vi "runDetectionB.vi"(0 "dl in":refnum<class "dl.lvclass">, 1 "batchSIze":i32=1, 2 "convert\nBGR2RGB":enum16{"False", "True"}(ring), 3 "BCHW":u16(ring)=1 items=["False", "True"], 4 "normalizeto255":enum16{"False", "True"}(ring), 5 "error in (no error)":errorcluster) -> (14 "dl out":refnum<class "dl.lvclass">, 15 "runSucc":i32, 16 "bbCounts":i32[](array[numeric]), 17 "maskCounts":i32[](array[numeric]), 19 "error out":errorcluster)   [LabVIEW 2025, in "dl.lvlib" / "dl.lvclass"]
doc: "Run Deep Learning Models – Bounding Box Detection and Segmentation**\n\nInputs:\n- `batchSize`: Number of input images (default: 1).\n- `BGR2RGB`: Convert image color format from BGR to RGB (default: false).\n- `BCHW`: Indicates whether the input is already in BCHW format (default: true).\n- `normalize255`: Normalize pixel values by dividing by 255 (default: false).\n\nOutputs:\n- `runSucc`: Algorithm execution status. `0` indicates success; any other value indicates an error.\n- `bbCounts`: Number of detected bounding boxes per image.\n- `maskCounts`: Number of detected segmentation masks per image."
uses:
  dl.lvclass
  dl.lvclass/dl.ctl
  e74e055a-5232-42f4-a9d8-d9d66c19bc29.vi
  0898d0a7-90d2-4c31-95aa-5e649e2e6c68.vi
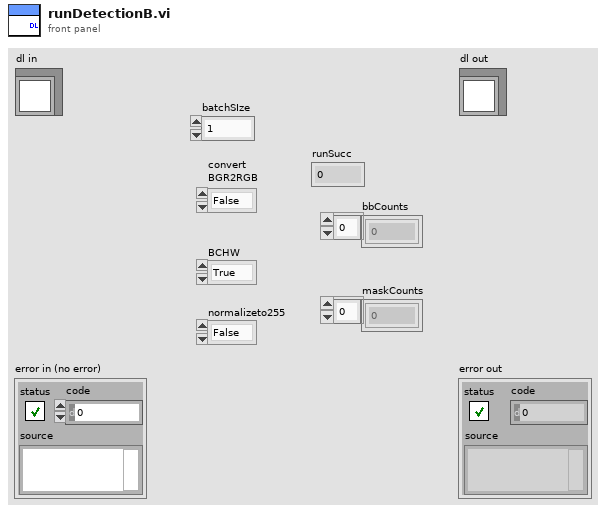
[diagram p1: front panel]
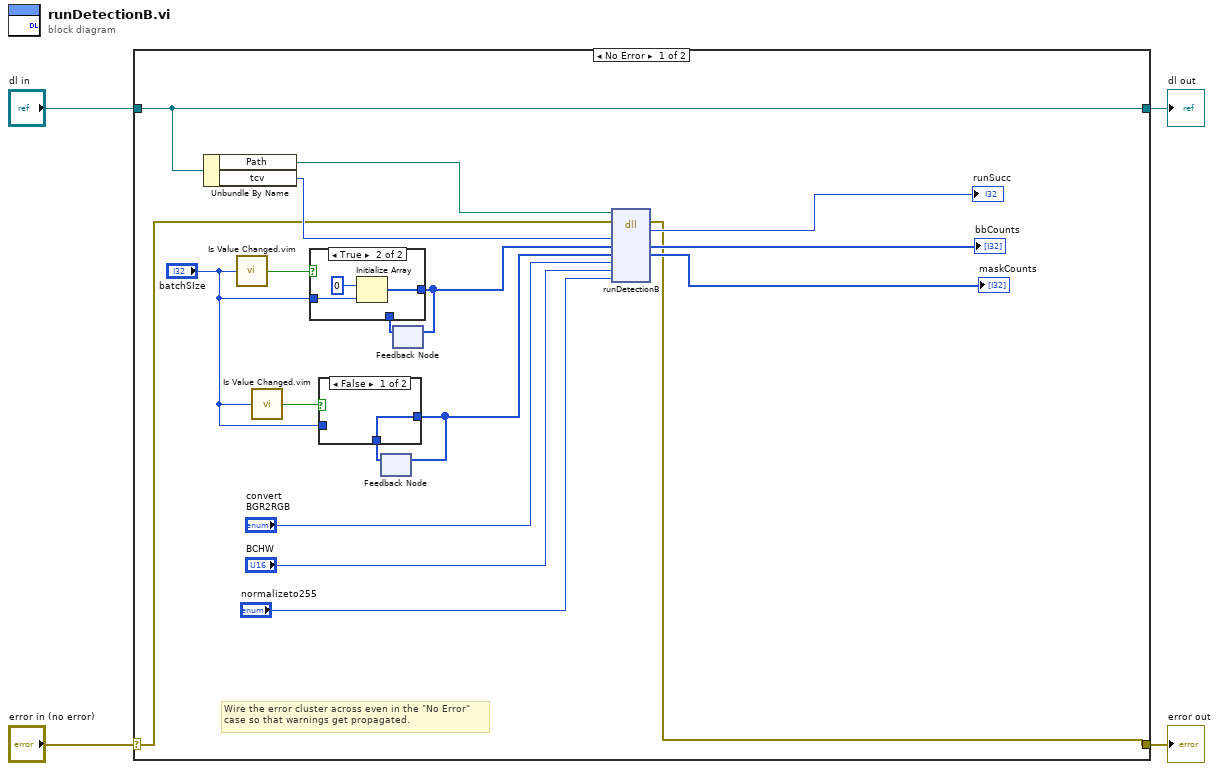
[diagram p0: block diagram]
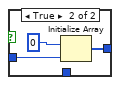
[diagram p2: hidden frame]
diagram:
  n1 = case shown="No Error" "error in (no error)" {
    selector: "error in (no error)" -> [w9 w32]
    tunnel: [w5 w32] -> w3
    tunnel: [w22 w31] -> w1
    tunnel: "dl in" -> [w22 w31]
    frame No Error {
      # "Wire the error cluster across even in the \"No Error\"\ncase so that warnings get propagated."
      n2 = Unbundle By Name(w22) -> ("Path"=w21:path, "tcv"=w20:u64)
      n3 = call "Is Value Changed.vim"("value"="batchSIze") -> ("changed or first call?"=w19:bool)
      n4 = call "Is Value Changed.vim"("value"="batchSIze") -> ("changed or first call?"=w16:bool)
      n5 = feedback #1() -> (w13:i32[])  [unwired: 1 in]
      n6 = case shown="False" w16 {
        tunnel: "batchSIze" -> [_ w26]
        tunnel: [w23 w24] -> w14
        tunnel: w13 -> [w23 _]
        frame False {
        }
        frame True {
          n7 = Initialize Array(0, w26) -> (w24:i32[])
        }
      }
      n8 = feedback-in #1(w14) -> ()
      n9 = feedback #2() -> (w17:i32[])  [unwired: 1 in]
      n10 = case shown="True" w19 {
        tunnel: "batchSIze" -> [_ w29]
        tunnel: [w27 w28] -> w18
        tunnel: w17 -> [w27 _]
        frame False {
        }
        frame True {
          n11 = Initialize Array(0, w29) -> (w28:i32[])
        }
      }
      n12 = feedback-in #2(w18) -> ()
      n13 = dll-call lib="D:/Test/adslvPackageDev/Resources/TCV_Lib.dll" fn="runDetectionB"(path in=w21, error in=w9, "tcv"=w20, "bbCounts"=w18, "maskCounts"=w14, "bgr2rgb"="convert\nBGR2RGB", "BCHW already"="BCHW", "normalizeto255"="normalizeto255") -> (error out=w5:errorcluster, "runSucc"=→"runSucc":i32, "bbCounts"=→"bbCounts":i32[], "maskCounts"=→"maskCounts":i32[])  [unwired: 5 in, 1 out]
    }
    frame Error {
    }
  }
  "error out" <- w3
  "dl out" <- w1
